vi "FLIR camera.vi"() -> ()   [LabVIEW 2025]
doc: "The Stream to AVI Files example shows how to save images to an AVI file when using a grab acquisition. This example uses a grab acquisition which works for all camera formats and image sizes. It is recommended to use the Stream to AVI File (Optimized Performance) example if your camera settings work with a ring acquisition."
uses:
  <vilib>/vision/driver/NI_Vision_Acquisition_Software.lvlib
  <resource>/objmgr/imaqdx.rc
  <vilib>/vision/Image Controls.llb/IMAQ Image.ctl
  VIs_needed/Grab Manager Mode.ctl
  <vilib>/vision/driver/IMAQdx.llb/IMAQdx Buffer Number Mode.ctl
  <vilib>/vision/Avi.llb/IMAQ AVI2 Codec Path.ctl
panel:
  out "Codec Speed (ms)":u32
  out "Boolean":bool
  out "Image Preview":T1(plugin-control)
  out "stripped path":path
  in  "Skip Count":u32
  out "Images Saved Per Second":dbl
  out "Images Acquired Per Second":dbl
  in  "Images per AVI":i32=100
  out "Write Speed":dbl(graph) caption="Image File Write Speed"
  in  "Start":bool
  in  "Codec":u16(ring) items=["FF Video Codec 1 (FFV1) (NI Vision)", "Motion JPEG (NI Vision)", "VP8 (NI Vision)", "VP9 (NI Vision)", "Y800 Uncompressed Grey Scale (NI Vision)", "YUV 4:2:0 Planar (NI Vision)"]
  out "Destination Folder":path
  out "Images Behind":i32
  in  "Number of Images":u32=30
  in  "Camera Name":refnum<k21> caption="IMAQdx Session"
  in  "Stop":bool
  # "Overview: Demonstrates how to stream images to an AVI file when using a grab acquisition.\nRequirements: Vision Acquisition Software\nInstructions:\n1. Select the Camera Name\n2. Run the VI\n3. Select the Codec and click Start.\n4. Increase the Skip Count if Images Behind is greater than 0."
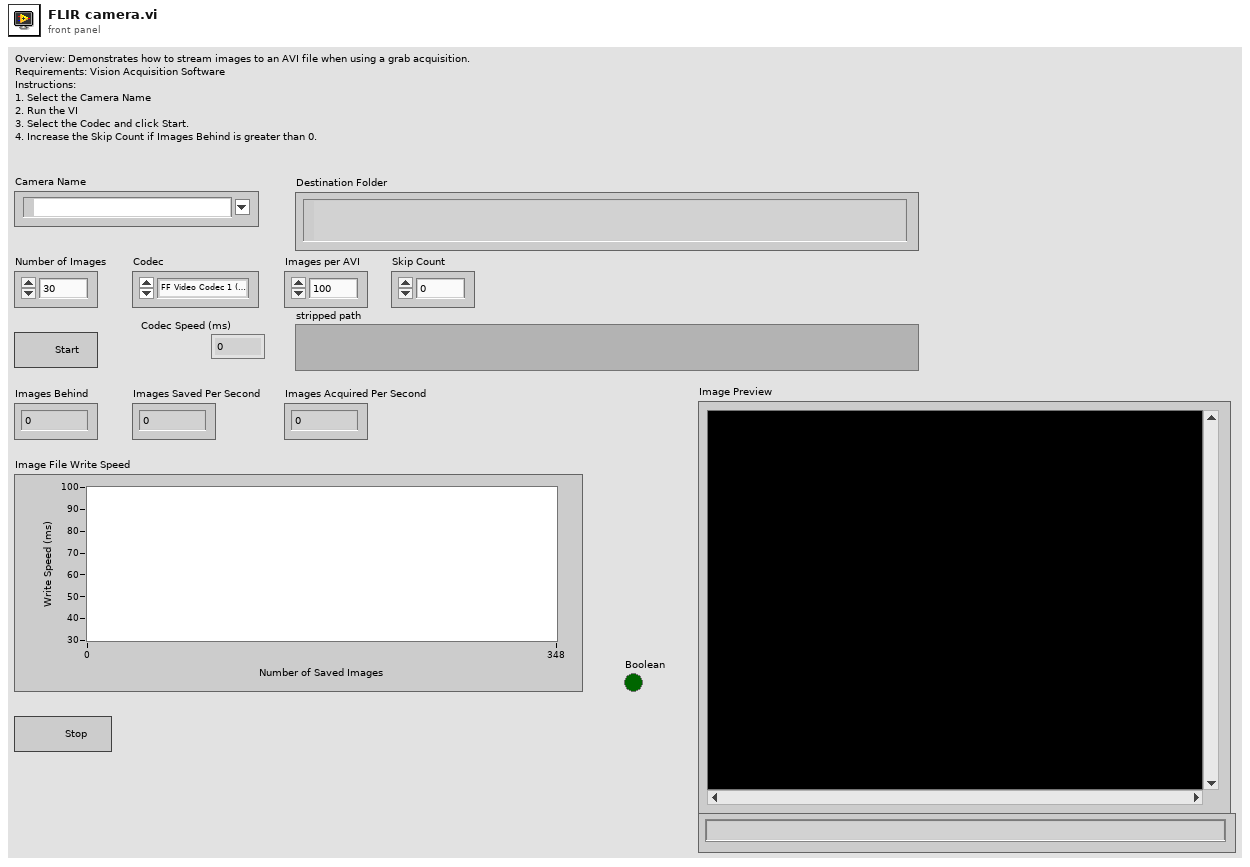
[diagram p1: front panel]
types:
  T1 = typedef "IMAQ Image.ctl" = refnum<image>
  T2 = typedef "IMAQ AVI2 Codec Path.ctl" = u32
  T3 = typedef "IMAQdx.ctl" = refnum<k21>
  T4 = typedef "Grab Manager Mode.ctl" = enum16{"Create Processing Images", "Lock", "Add Acquired Image", "Get Acquired Image", "Unlock", "Dispose Processing Images"}
  T5 = cluster{"Number of Processing Images":u32, "Image Border Size":u32}
  T6 = typedef "NI_Vision_Acquisition_Software.lvlib/IMAQdx Buffer Number Mode.ctl" = enum32{"Next", "Last", "Buffer Number", "Every", "Last New"}
  T7 = typedef "IMAQ AVI2 Refnum.ctl" = refnum<k20>
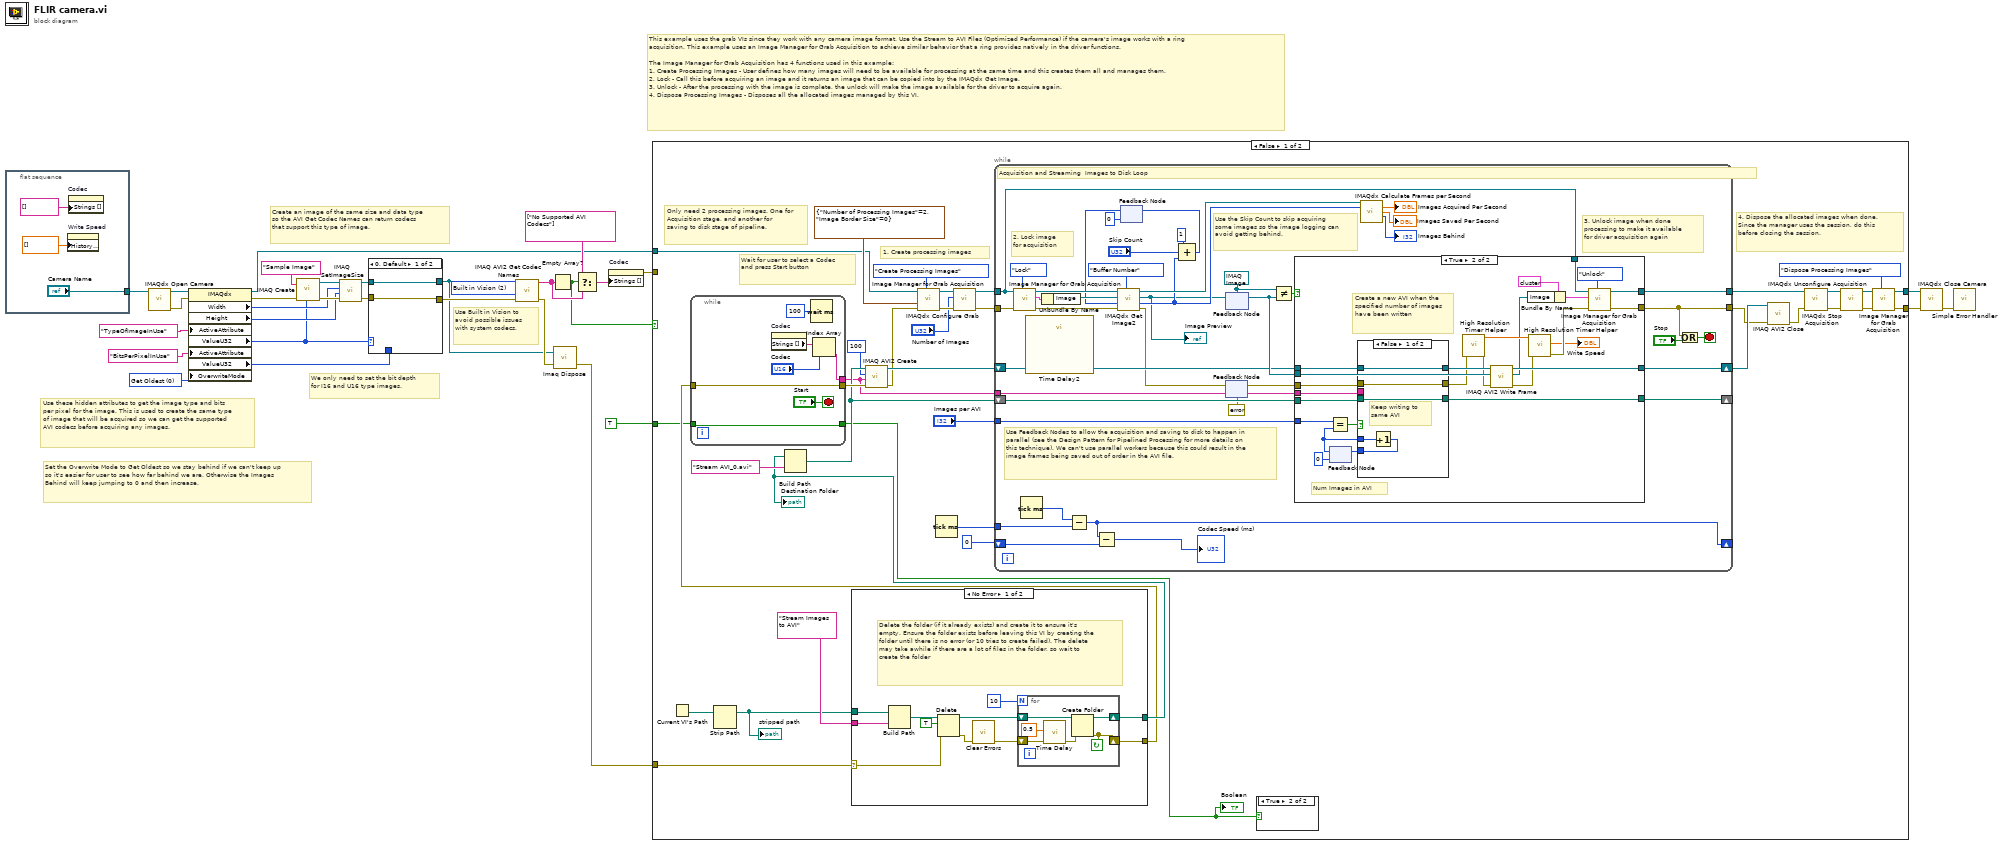
[diagram p0: block diagram]
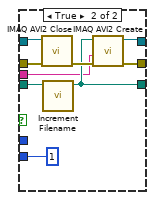
[diagram p5: hidden frame]
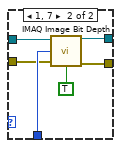
[diagram p7: hidden frame]
diagram:
  w2 = T2 2 items=["Default", "System", "Built in Vision"] ("Codec Source")
  w4 = u32 0 items=["Get Oldest"=0, "Fail"=2, "Get Newest"=3] ("OverwriteMode")
  # "Use Built in Vision to avoid possible issues with system codecs."
  # "This example uses the grab VIs since they work with any camera image format. Use the Stream to AVI Files (Optimized Performance) if the camera's image works with a ring acquisition. This example uses an Image Manager for Grab Acquisition to achieve similar behavior that a ring provides natively in the driver functions.\n\nThe Image Manager for Grab Acquisition has 4 functions used in this example:\n1. Create Processing Images - User defines how many images will need to be available for processing at the same time and this creates them all and manages them.\n2. Lock - Call this before acquiring an image and it returns an image that can be copied into by the IMAQdx Get Image.\n3. Unlock - After the processing with the image is complete, the unlock will make the image available for the driver to acquire again.\n4. Dispose Processing Images - Disposes all the allocated images managed by this VI."
  # "Set the Overwrite Mode to Get Oldest so we stay behind if we can't keep up so it's easier for user to see how far behind we are. Otherwise the Images Behind will keep jumping to 0 and then increase."
  # "Create an image of the same size and data type so the AVI Get Codec Names can return codecs that support this type of image."
  # "Use these hidden attributes to get the image type and bits per pixel for the image. This is used to create the same type of image that will be acquired so we can get the supported AVI codecs before acquiring any images."
  # "We only need to set the bit depth for I16 and U16 type images."
  n1 = flat-sequence {
    tunnel: ["Camera Name"] -> w31
    frame #0 {
      n2 = property on="Write Speed" class="WFChart (strict)"("History Data"=dbl[] []) -> ()  [unwired: 2 in, 2 out]
      n3 = property on="Codec" class="Ring (strict)"("Strings []"=string[] []) -> ()  [unwired: 2 in, 2 out]
    }
  }
  n4 = call <vilib>:"IMAQdx Open Camera.vi"("Session In"=w31) -> ("error out"=w27:errorcluster, "Session Out"=w28:T3)  [unwired: 2 in, 7 out]
  n5 = property class="IMAQdx"(reference=w28, error in=w27, "ActiveAttribute"="TypeOfImageInUse", "ActiveAttribute"="BitsPerPixelInUse", "OverwriteMode"=w4) -> (reference out=w13:T3, error out=w25:errorcluster, "Width"=w21:u32, "Height"=w20:u32, "ValueU32"=w8:u32, "ValueU32"=w11:u32)
  n6 = call "IMAQ Create"("Image Name"="Sample Image", "Image Type"=w8, "error in (no error)"=w25) -> ("New Image"=w22:T1, "error out"=w23:errorcluster)  [unwired: 1 in, 1 out]
  n7 = call "IMAQ SetImageSize"("error in (no error)"=w23, "Y Resolution"=w20, "X Resolution"=w21, "Image"=w22) -> ("error out"=w10:errorcluster, "Image Out"=w9:T1)  [unwired: 1 in]
  n8 = case shown="0, Default" w8 {
    tunnel: [w35 w42] -> w14
    tunnel: w11 -> [_ w41]
    tunnel: w10 -> [w35 w40]
    tunnel: w9 -> [w36 w38]
    tunnel: [w36 w37] -> w5
    frame 0, Default {
    }
    frame 1, 7 {
      n9 = call "IMAQ Image Bit Depth"("Image"=w38, "Bit Depth (0)"=w41, "error in (no error)"=w40, "Get/Set Bit Depth? (Set)"=TRUE) -> ("Image Out"=w37:T1, "error out"=w42:errorcluster)  [unwired: 9 in, 1 out]
    }
  }
  n10 = call "IMAQ AVI2 Get Codec Names"("error in (no error)"=w14, "Codec Source"=w2, "Image"=w5) -> ("error out"=w7:errorcluster, "Codec Names"=w19:string[])  [unwired: 7 in]
  n11 = Empty Array?(array=w19) -> (empty?=w15:bool)
  n12 = call "Imaq Dispose"("Image"=w5, "error in (no error)"=w7) -> ("error out"=w6:errorcluster)  [unwired: 4 in]
  n13 = Select(t=string[] ["No Supported AVI Codecs"], s=w15, f=w19) -> (s? t:f=w17:string[])
  n14 = property on="Codec" class="Ring (strict)"("Strings []"=w17) -> (error out=w16:errorcluster)  [unwired: 2 in, 1 out]
  n15 = case shown="False" w15 {
    tunnel: [w55 w189] -> w30
    tunnel: [w56 w190] -> w29
    tunnel: w13 -> [w61 w190]
    tunnel: w6 -> [w52 w189]
    tunnel: w16 -> [_ _]
    tunnel: TRUE -> [w47 _]
    frame False {
      # "4. Dispose the allocated images when done. Since the manager uses the session, do this before closing the session."
      # "1. Create processing images"
      # "Only need 2 processing images. One for Acquisition stage, and another for saving to disk stage of pipeline."
      # "Wait for user to select a Codec and press Start button"
      n16 = Current VI's Path() -> (path=w49:path)
      n17 = Strip Path(path=w49) -> (stripped path=w48:path)  [unwired: 1 out]
      "stripped path" <- w48
      n18 = case shown="No Error" w52 {
        selector: w52 -> [w81 w97]
        tunnel: w48 -> [w90 _]
        tunnel: [w83 _] -> w51
        tunnel: "Stream Images to AVI" ("Folder Name") -> [w82 _]
        tunnel: [w80 w97] -> w50
        frame No Error {
          # "Delete the folder (if it already exists) and create it to ensure it's empty. Ensure the folder exists before leaving this VI by creating the folder until there is no error (or 10 tries to create failed). The delete may take awhile if there are a lot of files in the folder, so wait to create the folder"
          n19 = Build Path(base path=w90, name or relative path=w82) -> (appended path=w88:path)
          n20 = Delete(path (use dialog)=w88, entire hierarchy (F)=TRUE, error in=w81) -> (deleted path=w87:path, error out=w86:errorcluster)  [unwired: 2 in, 1 out]
          n21 = call <vilib>:"Clear Errors.vi"("error in (no error)"=w86) -> ("error out"=w85:errorcluster)  [unwired: 5 in, 1 out]
          n22 = for {
            N: 10 -> [_]
            shift-right: [w95] -> w83
            shift-left: w87 -> [w96]
            shift-right: [w94] -> w80
            shift-left: w85 -> [w93]
            stop <- w94 continue-if-true
            n23 = call "Time Delay"("error in (no error)"=w93, "Delay Time (s)"=0.5) -> ("error out"=w92:errorcluster)  [unwired: 9 in]
            n24 = Create Folder(path (use dialog)=w96, error in=w92) -> (created path=w95:path, error out=w94:errorcluster)  [unwired: 2 out]
          }
        }
        frame Error {
        }
      }
      "Destination Folder" <- w51
      n25 = while {
        tunnel: w50 -> [w187]
        tunnel: [w187] -> w76
        tunnel: [w184] -> w68
        tunnel: [w182] -> w46
        tunnel: w47 -> [w182]
        stop <- "Start" stop-if-true
        n26 = property on="Codec" class="Ring (strict)"() -> ("Strings []"=w185:string[])  [unwired: 2 in, 2 out]
        n27 = Wait (ms)(milliseconds to wait=u32 100) -> ()  [unwired: 1 out]
        n28 = Index Array(array=w185, index="Codec") -> (element=w184:string)
      }
      "Boolean" <- w46
      n29 = Build Path(base path=w51, name or relative path="Stream AVI_0.avi") -> (appended path=w69:path)
      n30 = call "IMAQ AVI2 Create"("error in (no error)"=w76, "Codec"=w68, "Frames Per Second"=u32 100, "AVI Path"=w69) -> ("error out"=w60:errorcluster, "AVI Refnum"=w71:T7)  [unwired: 6 in]
      n31 = call "Image Manager for Grab Acquisition.vi"("Mode"=Grab_Manager_Mode."Create Processing Images", "error in (no error)"=w60, "Init Settings"=T5 {"Number of Processing Images"=2, "Image Border Size"=0}, "Session In"=w61) -> ("error out"=w63:errorcluster, "Session Out"=w62:T3)  [unwired: 4 in, 2 out]
      n32 = Tick Count (ms)() -> (millisecond timer value=w44:u32)
      n33 = call <vilib>:"IMAQdx Configure Grab.vi"("error in"=w63, "Number of Buffers"="Number of Images", "Session In"=w62) -> ("error out"=w66:errorcluster, "Session Out"=w67:T3)  [unwired: 7 in]
      n34 = while {
        tunnel: w66 -> [w120]
        tunnel: w67 -> [w121]
        tunnel: [w135] -> w77
        tunnel: [w128] -> w74
        shift-right: [w136] -> w75
        shift-left: w71 -> [w127]
        tunnel: "Images per AVI" -> [w123]
        shift-right: [w124] -> _
        shift-left: w69 -> [w125]
        tunnel: w68 -> [w126]
        tunnel: w44 -> [w102]
        shift-right: [w99] -> _
        shift-left: u32 0 -> [w101]
        shift-right: _ -> [_]
        shift-left: _ -> [_]
        stop <- w130 stop-if-true
        w133 = T1 refnum ("Image Out")
        # "3. Unlock image when done processing to make it available for driver acquisition again"
        # "2. Lock image for acquisition"
        # "Use the Skip Count to skip acquiring some images so the image logging can avoid getting behind."
        # "Use Feedback Nodes to allow the acquisition and saving to disk to happen in parallel (see the Design Pattern for Pipelined Processing for more details on this technique). We can't use parallel workers because this could result in the image frames being saved out of order in the AVI file."
        # "Acquisition and Streaming  Images to Disk Loop"
        n35 = call "Image Manager for Grab Acquisition.vi"("Mode"=Grab_Manager_Mode."Lock", "error in (no error)"=w120, "Session In"=w121) -> ("error out"=w117:errorcluster, "Image Settings Out"=w115:cluster{"Image":T1, "Buffer Number":u32}, "Session Out"=w118:T3)  [unwired: 5 in, 1 out]
        n36 = Tick Count (ms)() -> (millisecond timer value=w103:u32)
        n37 = call "Time Delay2"() -> ()  [unwired: 11 in, 1 out]
        n38 = Unbundle By Name(w115) -> ("Image"=w114:T1)
        n39 = Subtract(x=w103, y=w102) -> (x-y=w99:u32)
        n40 = Subtract(x=w99, y=w101) -> (x-y=→"Codec Speed (ms)":u32)
        n41 = feedback #1(u32 0) -> (w111:u32)
        n42 = call <vilib>:"IMAQdx Get Image2.vi"("Buffer Number Mode (Next)"=IMAQdx_Buffer_Number_Mode."Buffer Number", "error in"=w117, "Buffer Number In"=w111, "Image In"=w114, "Session In"=w118) -> ("error out"=w113:errorcluster, "Buffer Number Out"=w107:u32, "Image Out"=w98:T1, "Session Out"=w112:T3)  [unwired: 3 in]
        "Image Preview" <- w98
        n43 = Compound Arithmetic op=ADD(u32 1, "Skip Count", w107) -> (w106:u32)
        n44 = feedback-in #1(w106) -> ()
        n45 = feedback-in #2(w113) -> ()
        n46 = feedback #2(errorcluster {"status"=FALSE, "code"=0, "source"=""} ("error out")) -> (w134:errorcluster)
        n47 = feedback-in #3(w98) -> ()
        n48 = feedback #3(w133) -> (w131:T1)
        n49 = Not Equal?(x=w133, y=w131) -> (x != y?=w132:bool)
        n50 = case shown="True" w132 {
          tunnel: w127 -> [w139 w162]
          tunnel: w131 -> [_ w156]
          tunnel: w134 -> [w140 w161]
          tunnel: [w139 w167] -> w136
          tunnel: [w141 w150] -> w135
          tunnel: w121 -> [w141 w147]
          tunnel: [w140 w149] -> w128
          tunnel: w126 -> [_ w160]
          tunnel: w125 -> [w138 w159]
          tunnel: [w138 w157] -> w124
          tunnel: w123 -> [_ w155]
          frame False {
            # "First iteration doesn't have valid image for this pipelined stage."
          }
          frame True {
            # "Create a new AVI when the specified number of images have been written"
            # "Num Images in AVI"
            n51 = feedback #4(0) -> (w166:i32)
            n52 = Equal?(x=w155, y=w166) -> (x = y?=w163:bool)
            n53 = case shown="False" w163 {
              tunnel: [w171 1] -> w165
              tunnel: w166 -> [w172 _]
              tunnel: w162 -> [w170 w179]
              tunnel: [w170 w176] -> w158
              tunnel: w159 -> [w168 w180]
              tunnel: w161 -> [w169 w178]
              tunnel: [w169 w175] -> w154
              tunnel: [w168 w174] -> w157
              tunnel: w160 -> [_ w173]
              frame False {
                # "Keep writing to same AVI"
                n54 = Increment(x=w172) -> (x+1=w171:i32)
              }
              frame True {
                n55 = call "IMAQ AVI2 Close"("error in (no error)"=w178, "AVI Refnum"=w179) -> ("error out"=w177:errorcluster)  [unwired: 9 in]
                n56 = call "Increment Filename.vi"("Path In"=w180) -> ("Incremented Path Out"=w174:path)  [unwired: 10 in]
                n57 = call "IMAQ AVI2 Create"("error in (no error)"=w177, "Codec"=w173, "AVI Path"=w174) -> ("error out"=w175:errorcluster, "AVI Refnum"=w176:T7)  [unwired: 7 in]
              }
            }
            n58 = feedback-in #4(w165) -> ()
            n59 = call "High Resolution Timer Helper.vi"("error in (no error)"=w154) -> ("error out"=w153:errorcluster, "Current Time"=w151:dbl)  [unwired: 8 in, 1 out]
            n60 = call "IMAQ AVI2 Write Frame"("error in (no error)"=w153, "Image"=w156, "AVI Refnum"=w158) -> ("error out"=w152:errorcluster, "Image Out (duplicate)"=w144:T1, "AVI Refnum (duplicate)"=w167:T7)  [unwired: 6 in]
            n61 = Bundle By Name(cluster=cluster{"Image":T1, "Buffer Number":u32} {"Image"=refnum, "Buffer Number"=0} ("Image Settings In"), "Image"=w144) -> (w143:cluster{"Image":T1, "Buffer Number":u32})
            n62 = call "High Resolution Timer Helper.vi"("error in (no error)"=w152, "Previous Time"=w151) -> ("error out"=w148:errorcluster, "Time Difference (ms)"=→"Write Speed":dbl)  [unwired: 7 in, 1 out]
            n63 = call "Image Manager for Grab Acquisition.vi"("Mode"=Grab_Manager_Mode."Unlock", "error in (no error)"=w148, "Image Settings In"=w143, "Session In"=w147) -> ("error out"=w149:errorcluster, "Session Out"=w150:T3)  [unwired: 4 in, 2 out]
          }
        }
        n64 = call <vilib>:"IMAQdx Calculate Frames per Second.vi"("Session In"=w112, "Buffer Number"=w107) -> ("Acquired Frames per Second"=→"Images Acquired Per Second":dbl, "Processed Frames per Second"=→"Images Saved Per Second":dbl, "Images Behind"=→"Images Behind":i32)  [unwired: 7 in, 4 out]
        n65 = Or(x=w128, y="Stop") -> (x .or. y?=w130:bool)
      }
      n66 = case shown="True" w46 {
        frame False {
        }
        frame True {
        }
      }
      n67 = call "IMAQ AVI2 Close"("error in (no error)"=w74, "AVI Refnum"=w75) -> ("error out"=w73:errorcluster)  [unwired: 9 in]
      n68 = call <vilib>:"IMAQdx Stop Acquisition.vi"("error in"=w73, "Session In"=w77) -> ("error out"=w78:errorcluster, "Session Out"=w79:T3)  [unwired: 8 out]
      n69 = call <vilib>:"IMAQdx Unconfigure Acquisition.vi"("error in"=w78, "Session In"=w79) -> ("error out"=w59:errorcluster, "Session Out"=w58:T3)  [unwired: 8 out]
      n70 = call "Image Manager for Grab Acquisition.vi"("Mode"=Grab_Manager_Mode."Dispose Processing Images", "error in (no error)"=w59, "Session In"=w58) -> ("error out"=w55:errorcluster, "Session Out"=w56:T3)  [unwired: 5 in, 2 out]
    }
    frame True {
      # "No valid AVI Codecs for the image size and image type."
    }
  }
  n71 = call <vilib>:"IMAQdx Close Camera.vi"("error in"=w30, "Session In"=w29) -> ("error out"=w3:errorcluster)  [unwired: 9 out]
  n72 = call <vilib>:"Simple Error Handler.vi"("error in (no error)"=w3) -> ()  [unwired: 4 in, 5 out]
